vi "Run_VI.vi"(0 "Path":path, 11 "Error In":errorcluster) -> (4 "VI Refnum":refnum<vi>, 15 "Error Out":errorcluster)   [LabVIEW 2026, in "Core.lvlib"]
doc: "This VI runs Subpanel VI."
uses:
  Core.lvlib
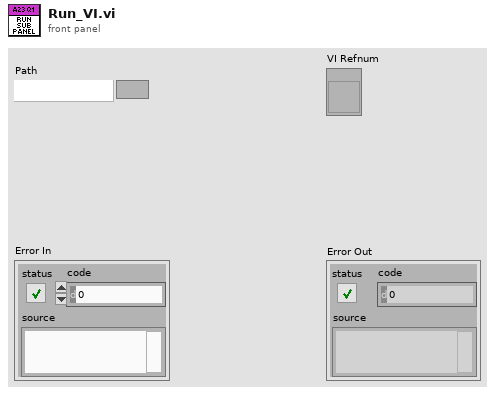
[diagram p1: front panel]
types:
  T1 = enum32{"Bad", "Idle", "Run top level", "Running"}
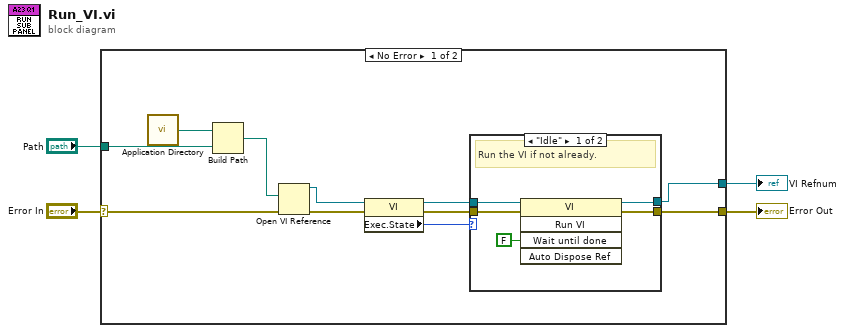
[diagram p0: block diagram]
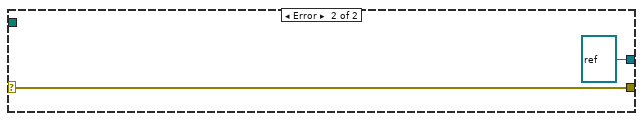
[diagram p3: hidden frame]
diagram:
  n1 = case shown="No Error" "Error In" {
    selector: "Error In" -> [w12 w24]
    tunnel: [w8 w24] -> w3
    tunnel: [w7 refnum<vi> refnum] -> w2
    tunnel: "Path" -> [w5 _]
    frame No Error {
      n2 = call <vilib>:"Application Directory.vi"() -> ("Application Directory"=w6:path)
      n3 = Build Path(base path=w6, name or relative path=w5) -> (appended path=w9:path)
      n4 = Open VI Reference(vi path=w9, error in (no error)=w12) -> (vi reference=w10:refnum<vi>, error out=w11:errorcluster)  [unwired: 4 in]
      n5 = property class="VI"(reference=w10, error in=w11) -> (reference out=w15:refnum<vi>, error out=w14:errorcluster, "Exec.State"=w13:T1)
      n6 = case shown="\"Idle\"" w13 {
        tunnel: w14 -> [w20 w21]
        tunnel: w15 -> [w18 w22]
        tunnel: [w19 w21] -> w8
        tunnel: [w17 w22] -> w7
        frame "Idle" {
          # "Run the VI if not already."
          n7 = invoke class="VI" method="Run VI"(reference=w18, error in=w20, "Wait until done"=FALSE ("Wait Until Done")) -> (reference out=w17:refnum<vi>, error out=w19:errorcluster)  [unwired: 2 in, 3 out]
        }
        frame Default {
          # "Continue."
        }
      }
    }
    frame Error {
    }
  }
  "Error Out" <- w3
  "VI Refnum" <- w2
